vi "Parse Status.vi"(4 "Status":string) -> (7 "Path Statuses":T1[](array[typedef]))   [LabVIEW 2020, in "VolatusGUI.lvlib" / "Git Updater Module.lvclass"]
uses:
  Git Updater Module.lvclass
  Path Status.ctl
  Status.ctl
  Git Updater Module.lvclass/Git Updater Module.ctl
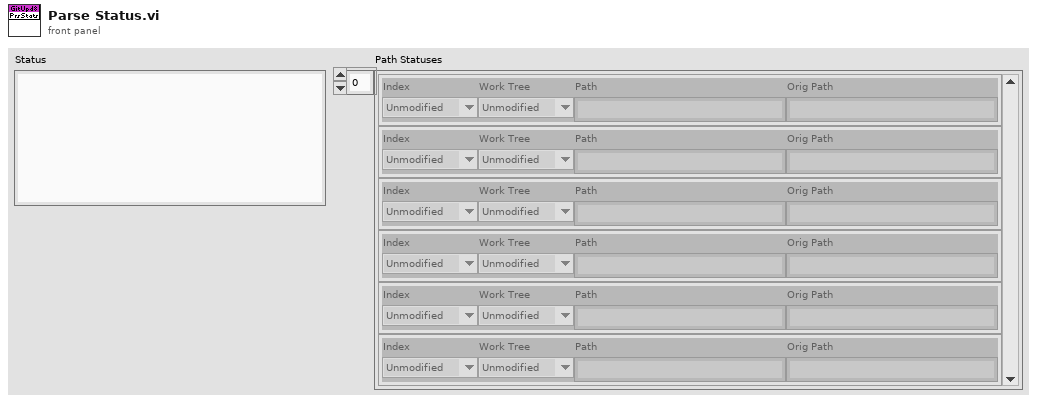
[diagram p1: front panel]
types:
  T1 = typedef "VolatusGUI.lvlib/Git Updater Module.lvclass/Path Status.ctl" = cluster{"Index":T2, "Work Tree":T2, "Path":string, "Orig Path":string}
  T2 = typedef "VolatusGUI.lvlib/Git Updater Module.lvclass/Status.ctl" = enum16{"UNKNOWN", "Unmodified", "Modified", "Added", "Deleted", "Renamed", "Unmerged", "Untracked", "Ignored"}
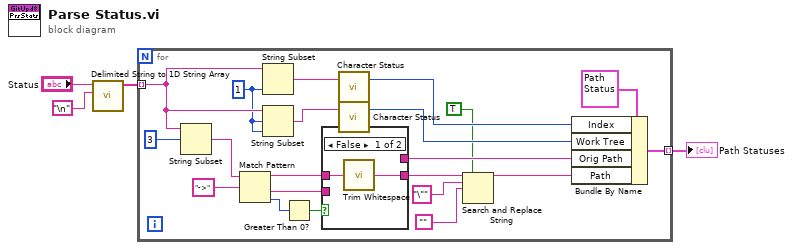
[diagram p0: block diagram]
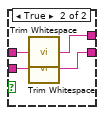
[diagram p2: hidden frame]
diagram:
  n1 = call <vilib>:"Delimited String to 1D String Array.vi"("delimiter"="\n", "delimited string"="Status") -> ("string array"=w2:string[])  [unwired: 9 in]
  n2 = for {
    tunnel: w2 -> [w13] mode=indexing
    tunnel: [w18] -> w1 mode=indexing
    w10 = 1 ("length (rest)")
    n3 = String Subset(string=w13, offset (0)=3) -> (substring=w11:string)  [unwired: 1 in]
    n4 = Match Pattern(string=w11, regular expression="->") -> (before substring=w21:string, after substring=w22:string, offset past match=w24:i32)  [unwired: 1 in, 1 out]
    n5 = String Subset(string=w13, length (rest)=w10) -> (substring=w15:string)  [unwired: 1 in]
    n6 = String Subset(string=w13, offset (0)=w10, length (rest)=w10) -> (substring=w17:string)
    n7 = Greater Than 0?(x=w24) -> (x > 0?=w23:bool)
    n8 = case shown="False" w23 {
      tunnel: w22 -> [_ w30]
      tunnel: w21 -> [w27 w31]
      tunnel: [w26 w29] -> w9
      tunnel: [_ w28] -> w19
      frame False {
        n9 = call <vilib>:"Trim Whitespace.vi"("string"=w27) -> ("trimmed string"=w26:string)  [unwired: 1 in]
      }
      frame True {
        n10 = call <vilib>:"Trim Whitespace.vi"("string"=w31) -> ("trimmed string"=w28:string)  [unwired: 1 in]
        n11 = call <vilib>:"Trim Whitespace.vi"("string"=w30) -> ("trimmed string"=w29:string)  [unwired: 1 in]
      }
    }
    n12 = call "Character Status.vi"("Character"=w15) -> ("Status"=w14:T2)  [unwired: 6 in]
    n13 = call "Character Status.vi"("Character"=w17) -> ("Status"=w16:T2)  [unwired: 6 in]
    n14 = Search and Replace String(replace all?=TRUE ("replace all? (F)"), input string=w9, search string="\"", replace string="") -> (result string=w5:string)  [unwired: 4 in, 3 out]
    n15 = Bundle By Name(cluster=T1 {"Index"=enum."Unmodified", "Work Tree"=enum."Unmodified", "Path"="", "Orig Path"=""} ("Path Status"), "Index"=w14, "Work Tree"=w16, "Orig Path"=w19, "Path"=w5) -> (w18:T1)
  }
  "Path Statuses" <- w1
